vi "MES_Flush.vi"(11 "Pending in":string[](array[string])) -> (0 "MES Error":errorcluster, 1 "Upload OK":bool, 2 "Pending Count":i32, 3 "Pending out":string[](array[string]), 5 "Upload Code":string)   [LabVIEW 2018]
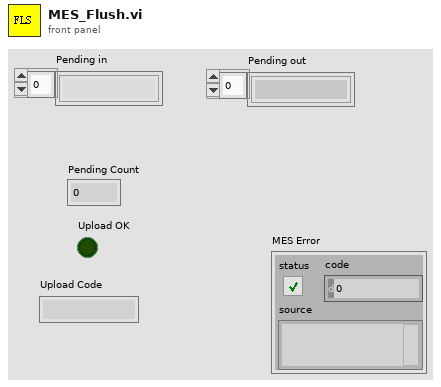
[diagram p1: front panel]
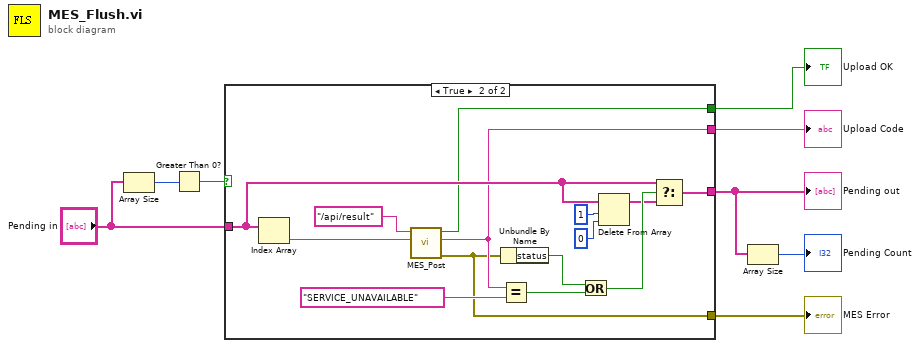
[diagram p0: block diagram]
diagram:
  n1 = Array Size(array="Pending in") -> (size(s)=w8:i32)
  n2 = Greater Than 0?(x=w8) -> (x > 0?=w7:bool)
  n3 = case shown="True" w7 {
    tunnel: "Pending in" -> [w9 w15]
    tunnel: [w9 w13] -> w2
    tunnel: [_ w12] -> w5
    tunnel: [_ w11] -> w4
    tunnel: [_ w10] -> w3
    frame False {
    }
    frame True {
      n4 = Index Array(array=w15) -> (element=w23:string)  [unwired: 1 in]
      n5 = call "MES_Post.vi"("Body"=w23, "Path"="/api/result") -> ("error out"=w10:errorcluster, "Code"=w11:string, "MES OK"=w12:bool)  [unwired: 6 in, 1 out]
      n6 = Unbundle By Name(w10) -> ("status"=w20:bool)
      n7 = Equal?(x=w11, y="SERVICE_UNAVAILABLE") -> (x = y?=w19:bool)
      n8 = Or(x=w20, y=w19) -> (x .or. y?=w16:bool)
      n9 = Delete From Array(array=w15, length=1, index=0) -> (array with subset deleted=w14:string[])  [unwired: 1 out]
      n10 = Select(t=w15, s=w16, f=w14) -> (s? t:f=w13:string[])
    }
  }
  "Pending out" <- w2
  "Upload OK" <- w5
  "Upload Code" <- w4
  "MES Error" <- w3
  n11 = Array Size(array=w2) -> (size(s)=→"Pending Count":i32)
